vi "GetSysColor Wrapper Template.vi"(0 "nIndex":i32=13, 11 "error in":errorcluster) -> (4 "color":u32, 15 "error out":errorcluster)   [LabVIEW 2020]
doc: "Returns the colour of a Windows display element through user32.dll GetSysColor (stdcall, called in any thread), as a COLORREF 0x00BBGGRR (red in the low byte). nIndex 13 COLOR_HIGHLIGHT is the background of a selected menu item. When error in carries an error the DLL is not called. Generated by tools\\Build Win32 Wrappers.vi - do not edit by hand, rebuild it."
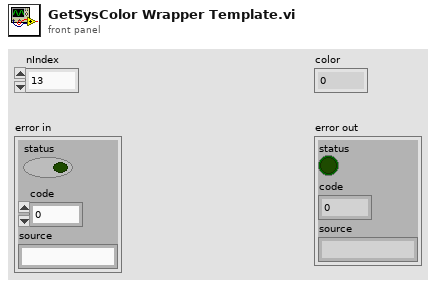
[diagram p1: front panel]
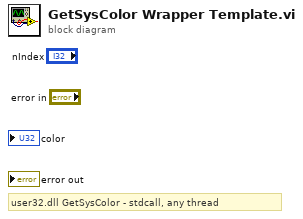
[diagram p0: block diagram]
diagram:
  # "user32.dll GetSysColor - stdcall, any thread"
